vi "Filter Task Rows.vi"(8 "error in":errorcluster, 10 "Show Inactive?":bool, 11 "Task Rows":T1[](array[typedef])) -> (0 "error out":errorcluster, 3 "Shown Rows":T1[](array[typedef]))   [LabVIEW 2026]
doc: "Returns the Task Edit Row clusters {Task Name, Active} to display: only the rows with Active TRUE while Show Inactive? is FALSE, every row while it is TRUE. Order is kept. Nothing is written - New Project.vi uses it to fill its Tasks control from its full task list.\n\nInputs: Task Rows; Show Inactive?; error in.\nOutputs: Shown Rows; error out (error in passed through).\n\nGenerated by: Claude"
uses:
  Task Edit Row.ctl
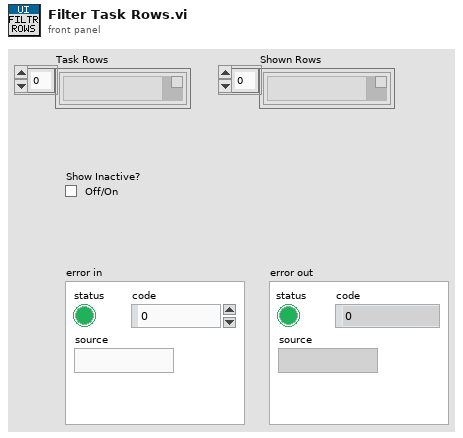
[diagram p1: front panel]
types:
  T1 = typedef "Task Edit Row.ctl" = cluster{"Task Name":string, "Active":bool}
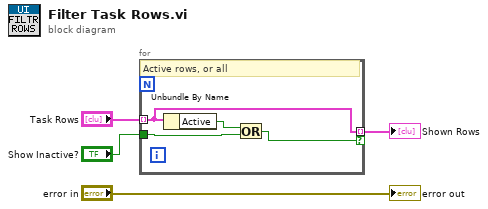
[diagram p0: block diagram]
diagram:
  n1 = for {
    tunnel: "Task Rows" -> [w5] mode=indexing
    tunnel: "Show Inactive?" -> [w6]
    tunnel: [w5] -> w4 mode=indexing if=w8
    # "Active rows, or all"
    n2 = Unbundle By Name(w5) -> ("Active"=w7:bool)
    n3 = Or(x=w7, y=w6) -> (x .or. y?=w8:bool)
  }
  "Shown Rows" <- w4
  "error out" <- "error in"
